vi "GOOP_GetOverlayIconPath.vi"(11 "IconName(NoPngExtension)":string) -> (3 "IconPath":path)   [LabVIEW 2020]
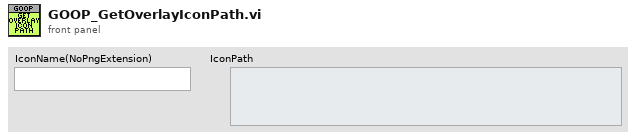
[diagram p1: front panel]
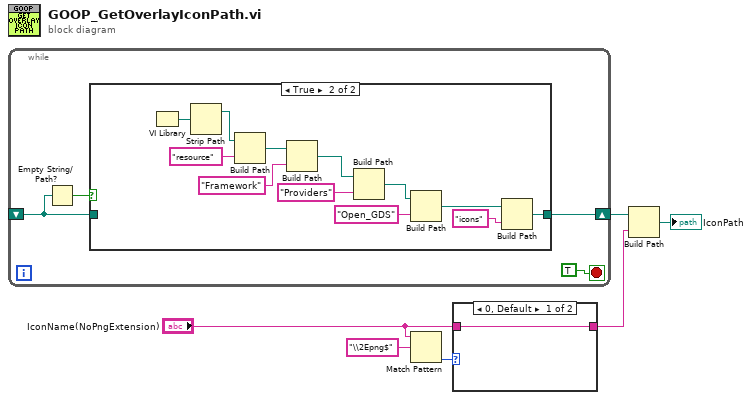
[diagram p0: block diagram]
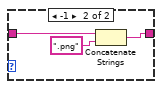
[diagram p2: hidden frame]
diagram:
  n1 = while {
    shift-right: [w9] -> w5
    shift-left: _ -> [w8]
    stop <- TRUE stop-if-true
    n2 = Empty String/Path?(string/path=w8) -> (empty?=w10:bool)
    n3 = case shown="True" w10 {
      tunnel: [w11 w13] -> w9
      tunnel: w8 -> [w11 _]
      frame False {
      }
      frame True {
        n4 = VI Library() -> (path=w15:path)
        n5 = Strip Path(path=w15) -> (stripped path=w16:path)  [unwired: 1 out]
        n6 = Build Path(base path=w16, name or relative path="resource") -> (appended path=w17:path)
        n7 = Build Path(base path=w17, name or relative path="Framework") -> (appended path=w18:path)
        n8 = Build Path(base path=w18, name or relative path="Providers") -> (appended path=w23:path)
        n9 = Build Path(base path=w23, name or relative path="Open_GDS") -> (appended path=w12:path)
        n10 = Build Path(base path=w12, name or relative path="icons") -> (appended path=w13:path)
      }
    }
  }
  n11 = Match Pattern(string="IconName(NoPngExtension)", regular expression="\\2Epng$" ("string")) -> (offset past match=w1:i32)  [unwired: 1 in, 3 out]
  n12 = case shown="0, Default" w1 {
    tunnel: [w24 w27] -> w6
    tunnel: "IconName(NoPngExtension)" -> [w24 w25]
    frame 0, Default {
    }
    frame -1 {
      n13 = Concatenate Strings(w25, ".png" ("string")) -> (w27:string)
    }
  }
  n14 = Build Path(base path=w5, name or relative path=w6) -> (appended path=→"IconPath":path)
